vi "Process.vi"(8 "error in":errorcluster, 11 "Plugin in":refnum<class "Nominal-TDMS-Upload.lvclass">) -> (0 "error out":errorcluster, 3 "Plugin out":refnum<class "Nominal-TDMS-Upload.lvclass">)   [LabVIEW 2020, in "Nominal-TDMS-Upload.lvlib" / "Nominal-TDMS-Upload.lvclass"]
uses:
  Nominal-TDMS-Upload.lvclass
  Nominal-TDMS-Upload.lvclass/Nominal-TDMS-Upload.ctl
  <vilib>/FlexLogger/SDK/PluginSDK.lvlibp/PEFClasses/SDK/System Interface/System Interface.lvclass
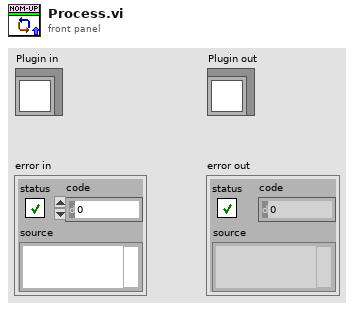
[diagram p1: front panel]
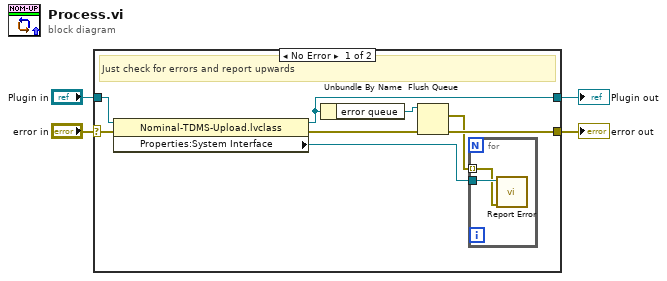
[diagram p0: block diagram]
diagram:
  n1 = case shown="No Error" "error in" {
    selector: "error in" -> [w11 w15]
    tunnel: [w7 w16] -> w1
    tunnel: "Plugin in" -> [w8 w16]
    tunnel: [w10 w15] -> w2
    frame No Error {
      # "Just check for errors and report upwards"
      n2 = property class="Nominal-TDMS-Upload.lvclass"(reference=w8, error in=w11) -> (reference out=w7:refnum<class "Nominal-TDMS-Upload.lvclass">, error out=w9:errorcluster, "Properties:System Interface"=w6:refnum<class "System Interface.lvclass">)
      n3 = Unbundle By Name(w7) -> ("error queue"=w12:refnum<queue>)
      n4 = Flush Queue(queue=w12, error in (no error)=w9) -> (remaining elements=w5:errorcluster[], error out=w10:errorcluster)  [unwired: 1 out]
      n5 = for {
        tunnel: w6 -> [w14]
        tunnel: w5 -> [w13] mode=indexing
        n6 = call-dynamic "Report Error.vi"("error in (no error)"=w13, "System Interface in"=w14) -> ()  [unwired: 8 in, 2 out]
      }
    }
    frame Error {
    }
  }
  "error out" <- w2
  "Plugin out" <- w1
